vi "Q18_Nested_Loops.vi"() -> ()   [LabVIEW 2018]
doc: "Use this template to build a VI to use as a subVI."
panel:
  out "Indexing + Last Value":dbl[](array[numeric])
  out "Indexing + Concatenating":dbl[](array[numeric])
  out "Indexing + Indexing":dbl[][](array[numeric])
  in  "Data In":dbl[][](array[numeric])
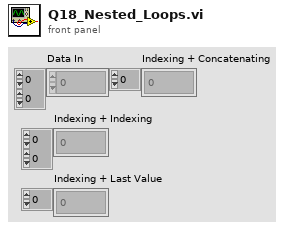
[diagram p1: front panel]
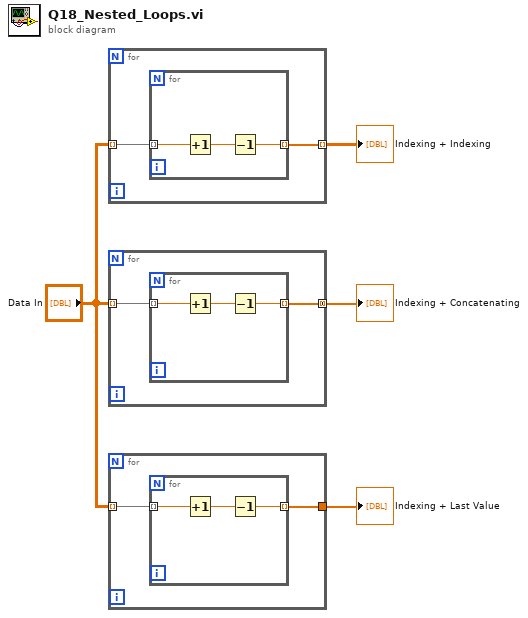
[diagram p0: block diagram]
diagram:
  n1 = for {
    tunnel: "Data In" -> [w6] mode=indexing
    tunnel: [w5] -> w4 mode=indexing
    n2 = for {
      tunnel: w6 -> [w9] mode=indexing
      tunnel: [w7] -> w5 mode=indexing
      n3 = Increment(x=w9) -> (x+1=w8:dbl)
      n4 = Decrement(x=w8) -> (x-1=w7:dbl)
    }
  }
  "Indexing + Indexing" <- w4
  n5 = for {
    tunnel: "Data In" -> [w11] mode=indexing
    tunnel: [w10] -> w3 mode=concatenating
    n6 = for {
      tunnel: w11 -> [w14] mode=indexing
      tunnel: [w12] -> w10 mode=indexing
      n7 = Increment(x=w14) -> (x+1=w13:dbl)
      n8 = Decrement(x=w13) -> (x-1=w12:dbl)
    }
  }
  "Indexing + Concatenating" <- w3
  n9 = for {
    tunnel: "Data In" -> [w16] mode=indexing
    tunnel: [w15] -> w1
    n10 = for {
      tunnel: w16 -> [w19] mode=indexing
      tunnel: [w17] -> w15 mode=indexing
      n11 = Increment(x=w19) -> (x+1=w18:dbl)
      n12 = Decrement(x=w18) -> (x-1=w17:dbl)
    }
  }
  "Indexing + Last Value" <- w1
